vi "RDV-GUI-SinglePlot.vi"() -> ()   [LabVIEW 2020]
doc: "Viewer, run by hand: loads all common-format files of a folder and shows reflection, impedance and permittivity on one graph. The user picks the folder and toggles which plots are visible."
uses:
  RDV-PRELAUNCH_DATA.ctl
  RDV-XY_GRAPH_REFS.ctl
  RDV-GUI_REFS.ctl
  RDV-PLOT_SETTINGS.ctl
  RDV-Reflection_Data_viewer.lvclass
panel:
  in  "imp imag":bool
  in  "imp real":bool
  in  "common name to remove":string="R140-"
  in  "Autoscale":bool
  in  "refl Imag":bool
  in  "refl Real":bool
  in  "Perm Imag":bool
  in  "Perm Real":bool
  in  "Toggle Plot":bool
  in  "Stop":bool
  out "error out":errorcluster
  in  "Folder Path":path=path "D:/projects/DielectricSpectroscopy/data/measurements/22p5c"
  out "Data":T1(graph)
  # "Reflection"
  # "Permativity"
  # "Impedance"
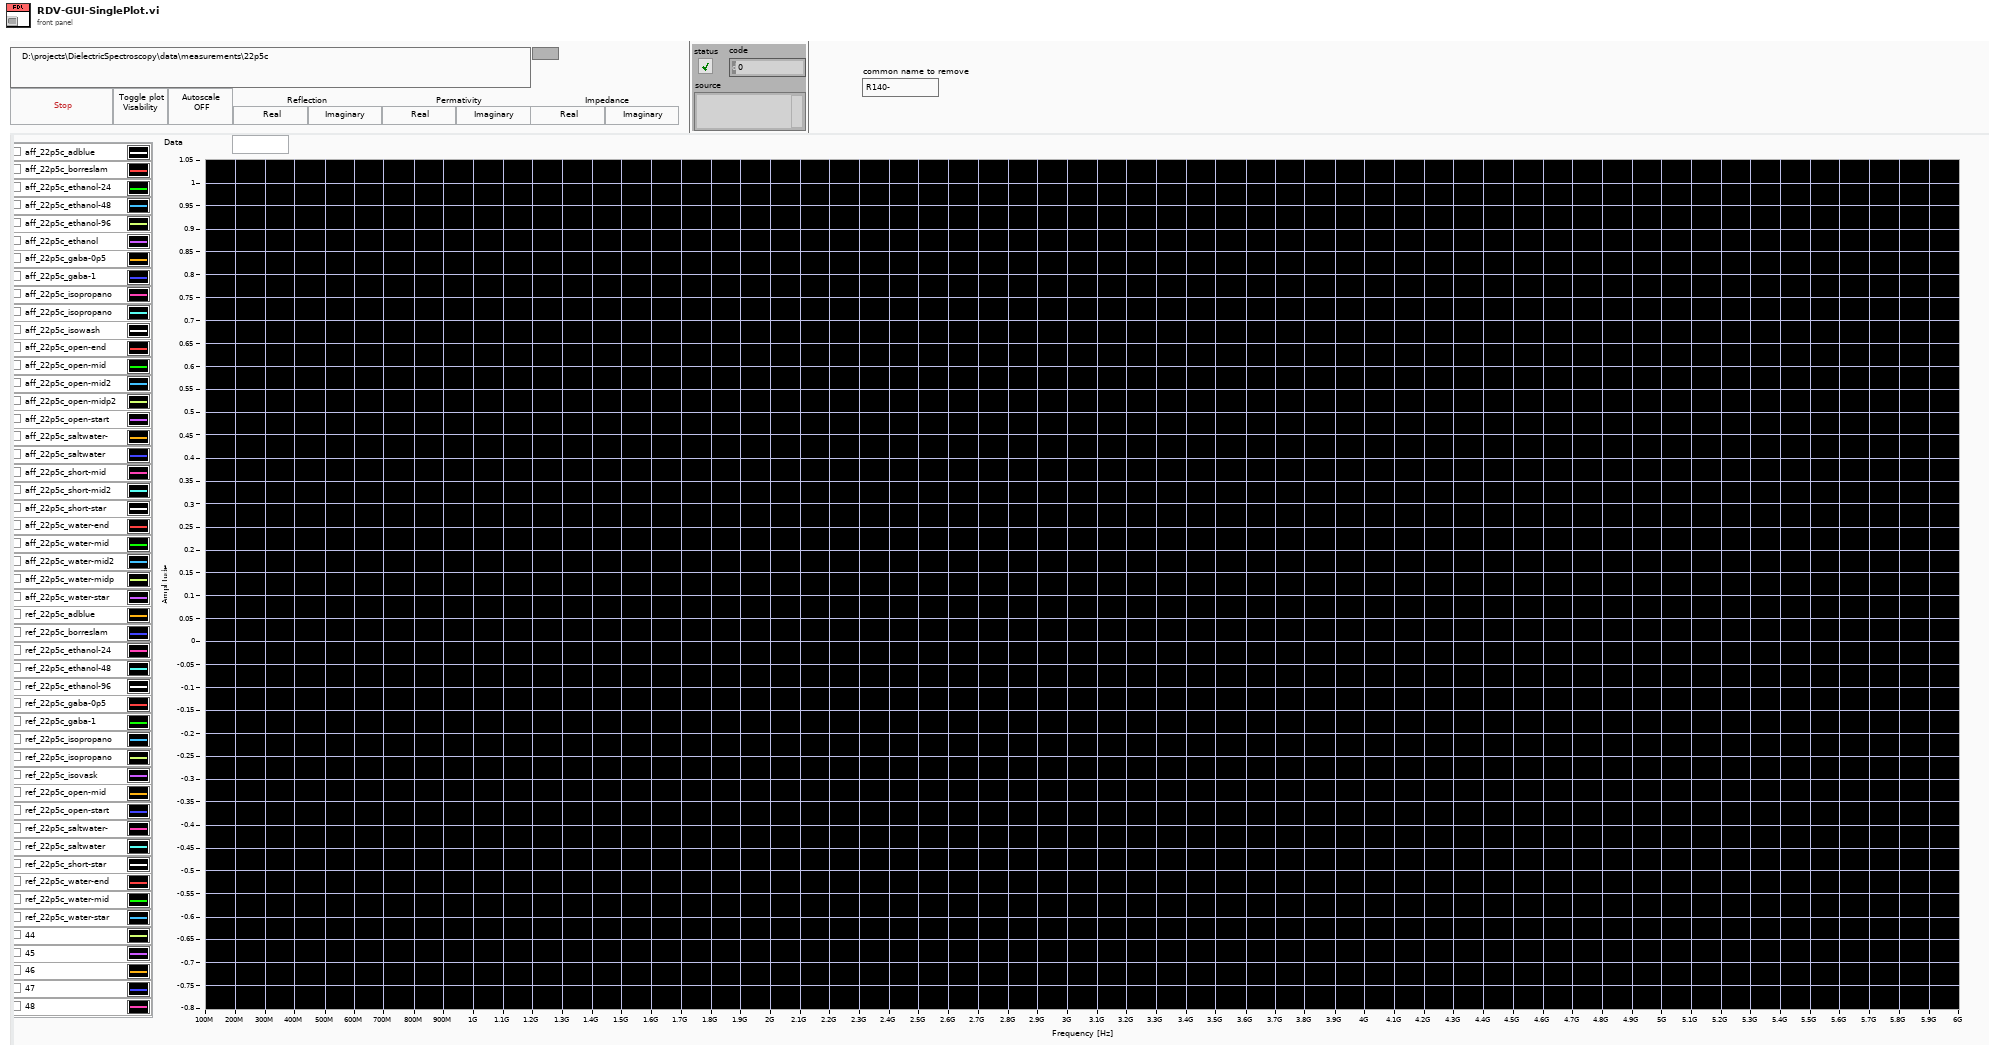
[diagram p1: front panel]
types:
  T1 = cluster{"Frequency":dbl[], "Reflection'":dbl[]}[]
  T2 = typedef "RDV-Reflection_Data_viewer.lvclass/RDV-PLOT_SETTINGS.ctl" = cluster{"common name to remove":string, "Max Size":i32}
  T3 = typedef "RDV-Reflection_Data_viewer.lvclass/RDV-PRELAUNCH_DATA.ctl" = cluster{"XY graph refs":T4, "GUI Refs":T5}
  T4 = typedef "RDV-Reflection_Data_viewer.lvclass/RDV-XY_GRAPH_REFS.ctl" = cluster{"Reflection Real":refnum<vi>, "Reflection Imag":refnum<vi>, "Permittivity Real":refnum<vi>, "Permittivity Imag":refnum<vi>, "Impedance Real":refnum<vi>, "Impedance Imag":refnum<vi>}
  T5 = typedef "RDV-Reflection_Data_viewer.lvclass/RDV-GUI_REFS.ctl" = cluster{"Autoscale":refnum<vi>, "sgl plot Selector":refnum<vi>[], "Smith Plot":refnum<vi>, "plot vis master ":refnum<vi>}
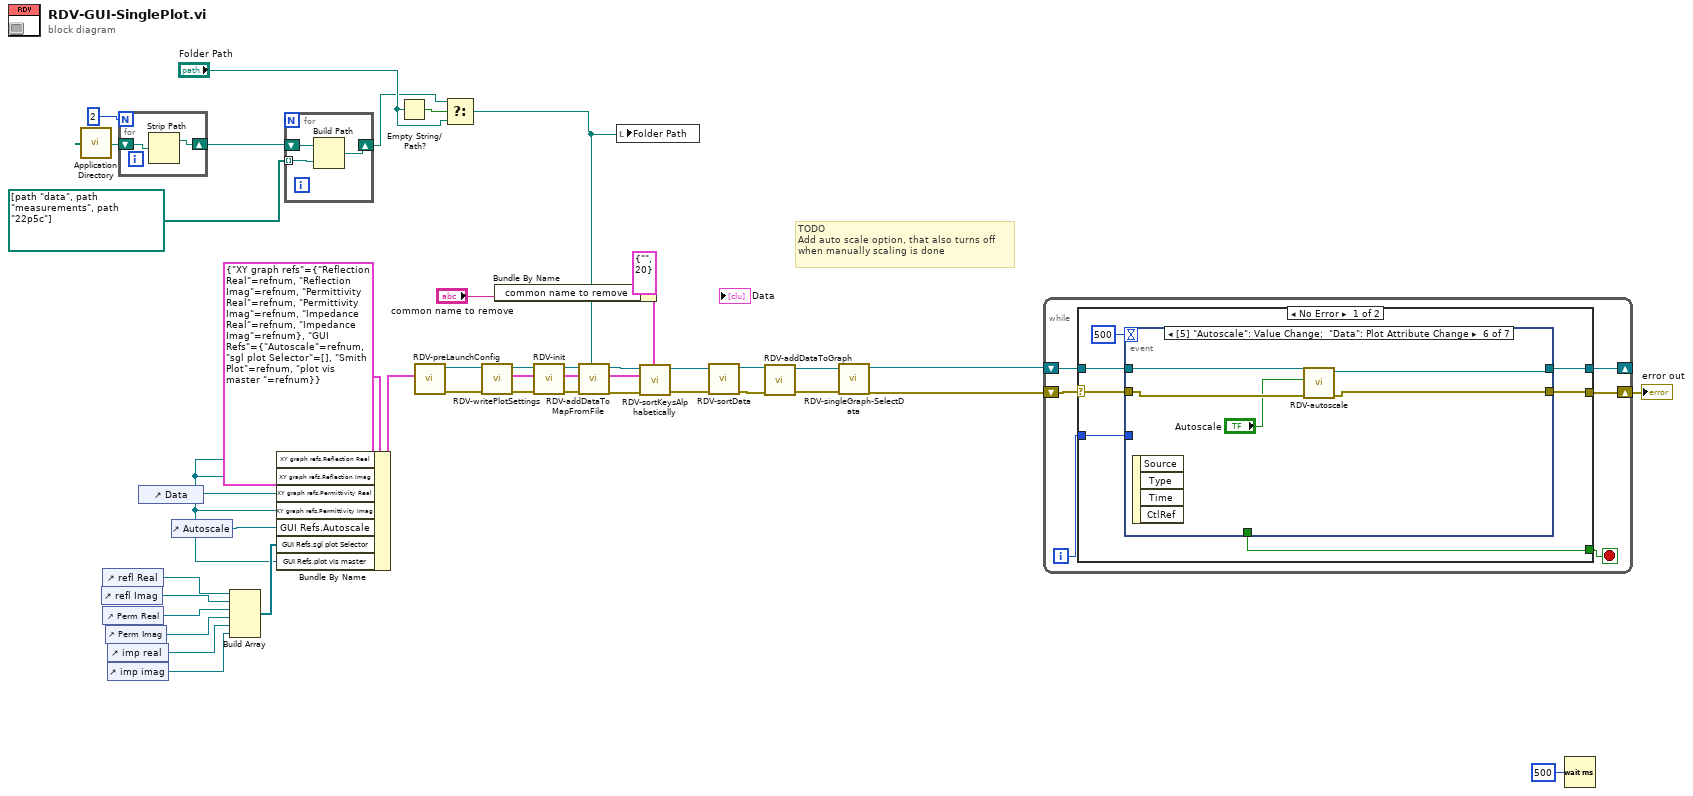
[diagram p0: block diagram]
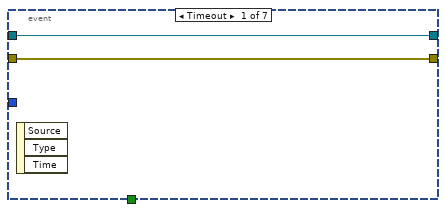
[diagram p2: hidden frame]
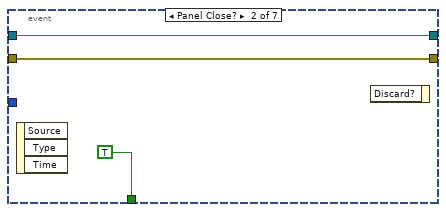
[diagram p3: hidden frame]
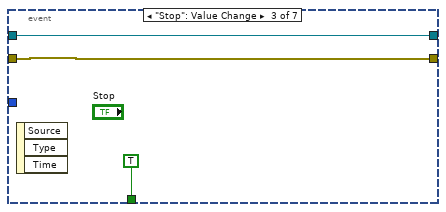
[diagram p4: hidden frame]
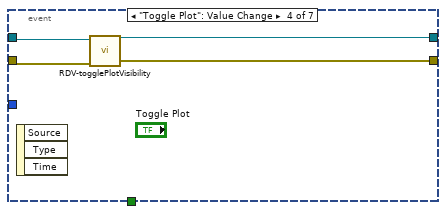
[diagram p5: hidden frame]
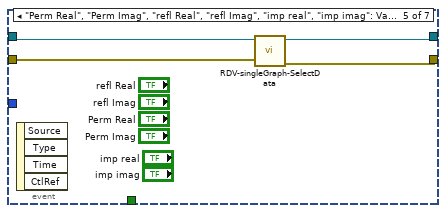
[diagram p6: hidden frame]
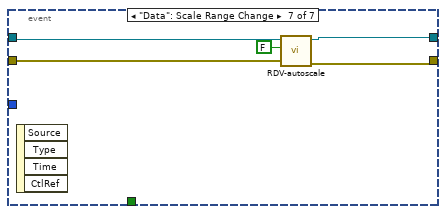
[diagram p7: hidden frame]
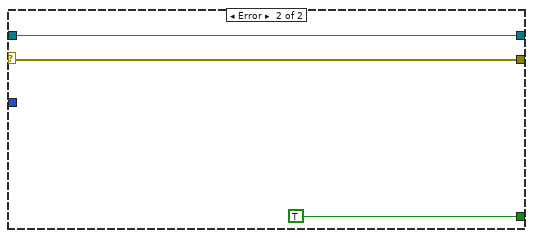
[diagram p8: hidden frame]
diagram:
  # "TODO\nAdd auto scale option, that also turns off\nwhen manually scaling is done"
  n1 = call <vilib>:"Application Directory.vi"() -> ("Application Directory"=w5:path)
  n2 = control-ref of="refl Imag"() -> (w21:refnum<vi>)
  n3 = control-ref of="refl Real"() -> (w22:refnum<vi>)
  n4 = control-ref of="Perm Real"() -> (w20:refnum<vi>)
  n5 = control-ref of="Perm Imag"() -> (w19:refnum<vi>)
  n6 = control-ref of="imp real"() -> (w10:refnum<vi>)
  n7 = control-ref of="imp imag"() -> (w9:refnum<vi>)
  n8 = for {
    N: 2 -> [_]
    shift-right: [w41] -> w4
    shift-left: w5 -> [w42]
    n9 = Strip Path(path=w42) -> (stripped path=w41:path)  [unwired: 1 out]
  }
  n10 = control-ref of="Data"() -> (w18:refnum<vi>)
  n11 = control-ref of="Autoscale"() -> (w24:refnum<vi>)
  n12 = Build Array(w22, w21, w20, w19, w10, w9) -> (w23:refnum<vi>[])
  n13 = Bundle By Name(cluster=T3 {"XY graph refs"={"Reflection Real"=refnum, "Reflection Imag"=refnum, "Permittivity Real"=refnum, "Permittivity Imag"=refnum, "Impedance Real"=refnum, "Impedance Imag"=refnum}, "GUI Refs"={"Autoscale"=refnum, "sgl plot Selector"=[], "Smith Plot"=refnum, "plot vis master "=refnum}} ("preLaunch Config"), "XY graph refs.Reflection Real"=w18, "XY graph refs.Reflection Imag"=w18, "XY graph refs.Permittivity Real"=w18, "XY graph refs.Permittivity Imag"=w18, "GUI Refs.Autoscale"=w24, "GUI Refs.sgl plot Selector"=w23, "GUI Refs.plot vis master"=w18) -> (w32:T3)
  n14 = for {
    shift-right: [w44] -> w3
    shift-left: w4 -> [w45]
    tunnel: path[] [path "data", path "measurements", path "22p5c"] ("Application Directory") -> [w43] mode=indexing
    n15 = Build Path(base path=w45, name or relative path=w43) -> (appended path=w44:path)
  }
  n16 = Empty String/Path?(string/path="Folder Path") -> (empty?=w8:bool)
  n17 = call "RDV-preLaunchConfig.vi"("preLaunch Config"=w32) -> ("error out"=w14:errorcluster, "RDV-Reflection_Data_viewer out"=w17:refnum<class "RDV-Reflection_Data_viewer.lvclass">)  [unwired: 9 in]
  n18 = Select(t=w3, s=w8, f="Folder Path") -> (s? t:f=w1:path)
  n19 = Bundle By Name(cluster=T2 {"common name to remove"="", "Max Size"=20} ("Plot Settings"), "common name to remove"="common name to remove") -> (w12:T2)
  n20 = call "RDV-writePlotSettings.vi"("error in (no error)"=w14, "Plot Settings"=w12, "RDV-Reflection_Data_viewer in"=w17) -> ("error out"=w15:errorcluster, "RDV-Reflection_Data_viewer out"=w16:refnum<class "RDV-Reflection_Data_viewer.lvclass">)  [unwired: 7 in]
  n21 = call "RDV-init.vi"("error in (no error)"=w15, "RDV-Reflection_Data_viewer in"=w16) -> ("error out"=w30:errorcluster, "RDV-Reflection_Data_viewer out"=w31:refnum<class "RDV-Reflection_Data_viewer.lvclass">)  [unwired: 8 in]
  n22 = call "RDV-addDataToMapFromFile.vi"("Folder Path"=w1, "error in (no error)"=w30, "RDV-Reflection_Data_viewer in"=w31) -> ("error out"=w34:errorcluster, "RDV-Reflection_Data_viewer out"=w40:refnum<class "RDV-Reflection_Data_viewer.lvclass">)  [unwired: 6 in, 1 out]
  n23 = local write "Folder Path"(w1) -> ()
  n24 = call "RDV-sortKeysAlphabetically.vi"("error in (no error)"=w34, "RDV-Reflection_Data_viewer in"=w40) -> ("error out"=w35:errorcluster, "RDV-Reflection_Data_viewer out"=w39:refnum<class "RDV-Reflection_Data_viewer.lvclass">)  [unwired: 7 in, 1 out]
  n25 = call "RDV-sortData.vi"("error in (no error)"=w35, "RDV-Reflection_Data_viewer in"=w39) -> ("error out"=w36:errorcluster, "RDV-Reflection_Data_viewer out"=w37:refnum<class "RDV-Reflection_Data_viewer.lvclass">)  [unwired: 8 in]
  n26 = call "RDV-addDataToGraph.vi"("error in (no error)"=w36, "RDV-Reflection_Data_viewer in"=w37) -> ("error out"=w25:errorcluster, "RDV-Reflection_Data_viewer out"=w28:refnum<class "RDV-Reflection_Data_viewer.lvclass">)  [unwired: 8 in]
  n27 = call "RDV-singleGraph-SelectData.vi"("error in (no error)"=w25, "RDV-Reflection_Data_viewer in"=w28) -> ("error out"=w26:errorcluster, "RDV-Reflection_Data_viewer out"=w27:refnum<class "RDV-Reflection_Data_viewer.lvclass">)  [unwired: 8 in]
  n28 = while {
    shift-right: [w50] -> _
    shift-left: w27 -> [w51]
    shift-right: [w48] -> w33
    shift-left: w26 -> [w49]
    i -> [w46]
    stop <- w47 stop-if-true
    n29 = case shown="No Error" w49 {
      selector: w49 -> [w55 w86]
      tunnel: w51 -> [w56 w87]
      tunnel: [w58 w87] -> w50
      tunnel: [w57 w86] -> w48
      tunnel: [w53 TRUE ("stop")] -> w47
      tunnel: w46 -> [w52 _]
      frame No Error {
        n30 = event shown="[5] \"Autoscale\": Value Change;  \"Data\": Plot Attribute Change" {
          selector: _ -> [_ _ _ _ _ _ _]
          dyn-events: _ -> [_ _ _ _ _ _ _]
          timeout: 500 -> [_ _ _ _ _ _ _]
          tunnel: [w60 w62 w65 w70 w74 w76 w84] -> w58
          tunnel: w56 -> [w60 w62 w65 w67 w73 w78 w83]
          tunnel: [w59 w61 w64 w69 w71 w77 w81] -> w57
          tunnel: w55 -> [w59 w61 w64 w68 w72 w79 w82]
          tunnel: [_ TRUE ("Discard?") TRUE ("Discard?") _ _ _ _] -> w53
          tunnel: w52 -> [_ _ _ _ _ _ _]
          event Timeout {
            n31 = event-data() -> ()  [unwired: 1 in, 3 out]
          }
          event Panel Close? {
            n32 = event-data() -> ()  [unwired: 1 in, 3 out]
            n33 = event-data() -> ()  [unwired: 2 in, 1 out]
          }
          event "Stop": Value Change {
            n34 = event-data() -> ()  [unwired: 1 in, 3 out]
          }
          event "Toggle Plot": Value Change {
            n35 = event-data() -> ()  [unwired: 1 in, 3 out]
            n36 = call "RDV-togglePlotVisibility.vi"("error in (no error)"=w68, "RDV-Reflection_Data_viewer in"=w67) -> ("error out"=w69:errorcluster, "RDV-Reflection_Data_viewer out"=w70:refnum<class "RDV-Reflection_Data_viewer.lvclass">)  [unwired: 8 in]
          }
          event "Perm Real", "Perm Imag", "refl Real", "refl Imag", "imp real", "imp imag": Value Change {
            n37 = event-data() -> ()  [unwired: 1 in, 4 out]
            n38 = call "RDV-singleGraph-SelectData.vi"("error in (no error)"=w72, "RDV-Reflection_Data_viewer in"=w73) -> ("error out"=w71:errorcluster, "RDV-Reflection_Data_viewer out"=w74:refnum<class "RDV-Reflection_Data_viewer.lvclass">)  [unwired: 8 in]
          }
          event "Autoscale": Value Change; "Data": Plot Attribute Change {
            n39 = event-data() -> ()  [unwired: 1 in, 4 out]
            n40 = call "RDV-autoscale.vi"("error in (no error)"=w79, "Autoscale"="Autoscale", "RDV-Reflection_Data_viewer in"=w78) -> ("error out"=w77:errorcluster, "RDV-Reflection_Data_viewer out"=w76:refnum<class "RDV-Reflection_Data_viewer.lvclass">)  [unwired: 7 in]
          }
          event "Data": Scale Range Change {
            n41 = event-data() -> ()  [unwired: 1 in, 4 out]
            n42 = call "RDV-autoscale.vi"("error in (no error)"=w82, "Autoscale"=FALSE, "RDV-Reflection_Data_viewer in"=w83) -> ("error out"=w81:errorcluster, "RDV-Reflection_Data_viewer out"=w84:refnum<class "RDV-Reflection_Data_viewer.lvclass">)  [unwired: 7 in]
          }
        }
      }
      frame Error {
      }
    }
  }
  "error out" <- w33
  n43 = Wait (ms)(milliseconds to wait=u32 500) -> ()  [unwired: 1 out]
